vi "随机二维数组.vi"() -> (0 "数组":i16[][](array[numeric]))   [LabVIEW 2017]
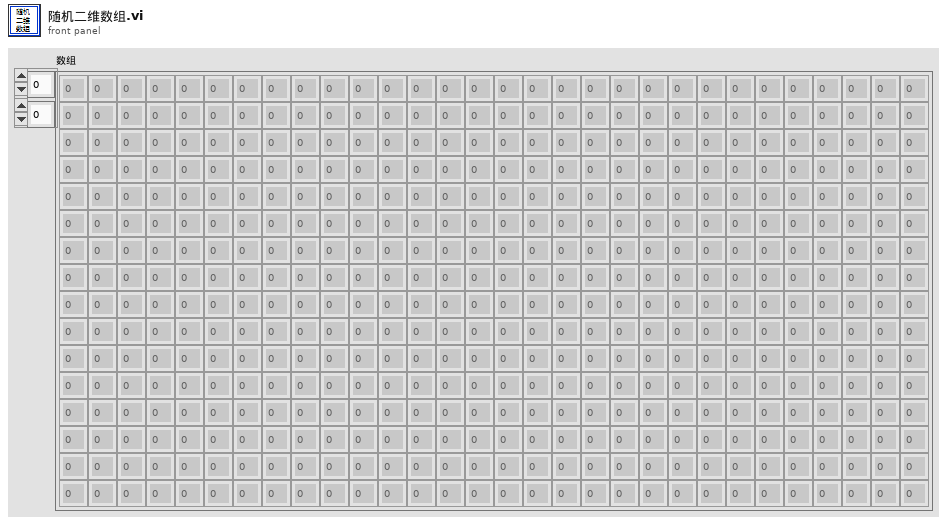
[diagram p1: front panel]
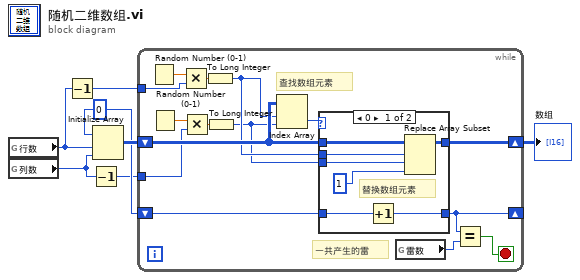
[diagram p0: block diagram]
diagram:
  w3 = 0
  n1 = global read "全局变量.vi" "行数"() -> (w4:i32)
  n2 = global read "全局变量.vi" "列数"() -> (w5:i32)
  n3 = Decrement(x=w4) -> (x-1=w2:i32)
  n4 = Decrement(x=w5) -> (x-1=w1:i32)
  n5 = Initialize Array(w3, w4, w5) -> (w6:i32[][])
  n6 = while {
    shift-right: [w16] -> w7
    shift-left: w6 -> [w19]
    tunnel: w1 -> [w8]
    tunnel: w2 -> [w12]
    shift-right: [w10] -> _
    shift-left: w3 -> [w11]
    stop <- w15 stop-if-true
    # "查找数组元素"
    # "一共产生的雷"
    n7 = Random Number (0-1)() -> (number: 0 to 1=w20:dbl)
    n8 = Random Number (0-1)() -> (number: 0 to 1=w9:dbl)
    n9 = Multiply(x=w20, y=w12) -> (x*y=w21:dbl)
    n10 = Multiply(x=w9, y=w8) -> (x*y=w22:dbl)
    n11 = To Long Integer(number=w21) -> (32bit integer=w18:i32)
    n12 = To Long Integer(number=w22) -> (32bit integer=w17:i32)
    n13 = Index Array(array=w19, index (row)=w18, index (col)=w17) -> (element=w14:i32)
    n14 = case shown="0" w14 {
      tunnel: [w29 w31] -> w16
      tunnel: w19 -> [w28 w31]
      tunnel: w18 -> [w27 _]
      tunnel: w17 -> [w26 _]
      tunnel: w11 -> [w24 w30]
      tunnel: [w23 w30] -> w10
      frame 0 {
        # "替换数组元素"
        n15 = Increment(x=w24) -> (x+1=w23:i32)
        n16 = Replace Array Subset(array=w28, new element=1, index (row)=w27, index (col)=w26) -> (w29:i32[][])
      }
      frame 1, Default {
      }
    }
    n17 = global read "全局变量.vi" "雷数"() -> (w13:i32)
    n18 = Equal?(x=w10, y=w13) -> (x = y?=w15:bool)
  }
  "数组" <- w7
